vi "edit io channel.vi"(8 "error in":errorcluster, 9 "line":T1, 10 "engine configuration in":refnum<class "engine configuration.lvclass">, 11 "tag bus configurable plugin module configuration in":refnum<class "Modbus Module configuration.lvclass">) -> (0 "error out":errorcluster, 1 "Change":bool, 2 "engine configuration":refnum<class "engine configuration.lvclass">, 3 "tag bus configurable plugin module configuration out":refnum<class "Modbus Module configuration.lvclass">)   [LabVIEW 2015, in "Modbus Module editor node.lvclass"]
doc: "Platypus Framework 1.0.1.65\nNI Systems Engineering - National Instruments"
uses:
  Modbus Module editor node.lvclass
  <vilib>/NI/Module Execution Interface/Engine Configuration/engine configuration.lvclass
  module/configuration/Modbus Module configuration.lvclass
  table line.ctl
  module/module channel/Modbus Module Channel.lvclass
  <vilib>/NI/Configuration Framework/serializable configuration/NISE_CEF_serializable configuration.lvclass/NISE_CEF_serializable configuration.ctl
  <vilib>/NI/Tag Bus/tag/tag descriptor.lvclass/tag descriptor.ctl
  <vilib>/Utility/LVClass/Get LV Class Name.vi
  <vilib>/NI/Configuration Framework/error generator/NISE_error generator.vi
  <vilib>/NI/Tag Bus/tag/tag descriptor.lvclass
  <vilib>/NI/Configuration Framework/serializable configuration/NISE_CEF_serializable configuration.lvclass
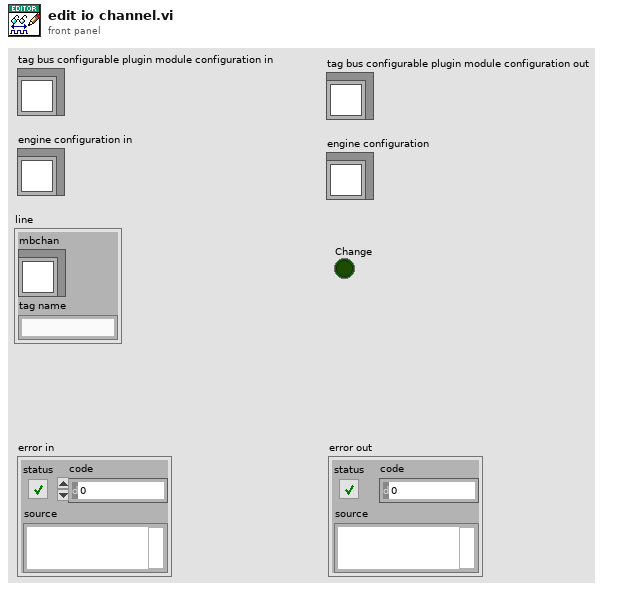
[diagram p1: front panel]
types:
  T1 = typedef "Modbus Module editor node.lvclass/table line.ctl" = cluster{"mbchan":refnum<class "Modbus Module Channel.lvclass">, "tag name":string}
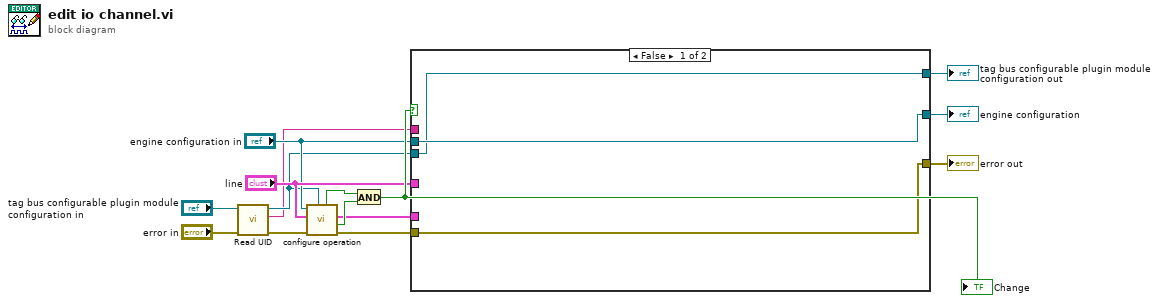
[diagram p0: block diagram]
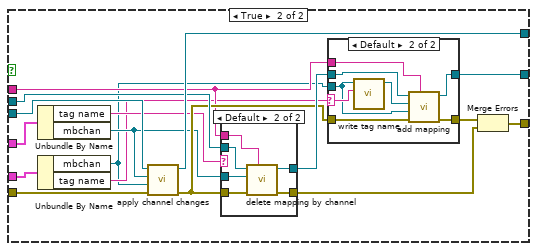
[diagram p2: hidden frame]
diagram:
  n1 = call <vilib>:"Read UID.vi"("error in"="error in", "configuration in"="tag bus configurable plugin module configuration in") -> ("error out"=w4:errorcluster, "instance id"=w1:string, "configuration out"=w2:refnum<class "Modbus Module configuration.lvclass">)  [unwired: 7 in]
  n2 = call "configure operation.vi"("tag bus configurable plugin module configuration"=w2, "error in"=w4, "line item in"="line", "engine configuration"="engine configuration in") -> ("error out"=w8:errorcluster, "success"=w12:bool, "line item out"=w9:T1, "changed"=w11:bool)  [unwired: 4 in]
  n3 = And(x=w11, y=w12) -> (x .and. y?=w13:bool)
  "Change" <- w13
  n4 = case shown="False" w13 {
    tunnel: [w17 w25] -> w6
    tunnel: [w18 w28] -> w15
    tunnel: "engine configuration in" -> [w18 w30]
    tunnel: w8 -> [w17 w32]
    tunnel: w9 -> [_ w34]
    tunnel: "line" -> [_ w33]
    tunnel: w2 -> [w16 w35]
    tunnel: [w16 w31] -> w14
    tunnel: w1 -> [_ w21]
    frame False {
    }
    frame True {
      n5 = Unbundle By Name(w33) -> ("tag name"=w23:string, "mbchan"=w22:refnum<class "Modbus Module Channel.lvclass">)
      n6 = Unbundle By Name(w34) -> ("mbchan"=w19:refnum<class "Modbus Module Channel.lvclass">, "tag name"=w20:string)
      n7 = call "apply channel changes.vi"("error in"=w32, "new channel"=w19, "old channel"=w22, "Modbus Slave configuration in"=w35) -> ("error out"=w24:errorcluster, "Modbus Slave configuration out"=w31:refnum<class "Modbus Module configuration.lvclass">)  [unwired: 6 in]
      n8 = case shown="Default" w23 {
        tunnel: w21 -> [_ w53]
        tunnel: w30 -> [w47 w52]
        tunnel: [w47 w51] -> w29
        tunnel: [w46 w50] -> w27
        tunnel: w24 -> [w46 w49]
        tunnel: w22 -> [_ w48]
        frame "" {
        }
        frame Default {
          n9 = call <vilib>:"delete mapping by channel.vi"("owner ID"=w53, "error in"=w49, "channel"=w48, "engine configuration in"=w52) -> ("error out"=w50:errorcluster, "engine configuration out"=w51:refnum<class "engine configuration.lvclass">)  [unwired: 6 in]
        }
      }
      n10 = case shown="Default" w20 {
        selector: w20 -> [_ w39]
        tunnel: w29 -> [w37 w45]
        tunnel: [w37 w44] -> w28
        tunnel: [w36 w43] -> w26
        tunnel: w24 -> [w36 w42]
        tunnel: w21 -> [_ w41]
        tunnel: w19 -> [_ w38]
        frame "" {
        }
        frame Default {
          n11 = call <vilib>:"write tag name.vi"("name"=w39, "system tag in"=w38) -> ("system tag out"=w40:refnum<class "Modbus Module Channel.lvclass">)  [unwired: 8 in, 1 out]
          n12 = call-dynamic "add mapping.vi"("owner ID"=w41, "error in"=w42, "channel"=w38, "tag descriptor"=w40, "engine configuration"=w45) -> ("error out"=w43:errorcluster, "engine configuration out"=w44:refnum<class "engine configuration.lvclass">)  [unwired: 5 in]
        }
      }
      n13 = Merge Errors(w26, w27) -> (w25:errorcluster)
    }
  }
  "engine configuration" <- w15
  "tag bus configurable plugin module configuration out" <- w14
  "error out" <- w6
